vi "Stewart_platform_6_deg_freedom_ver4_easier_upgrade.vi"() -> ()   [LabVIEW 2019]
uses:
  SubVI/Type_definition_updated_motion_output_row.ctl
  SubVI/Type_definition_current_motion.ctl
  SubVI/Type_definition.ctl
panel:
  out "結果":bool
  in  "One way control":T1={"T"=2000.0, "Linear or sine?"=0.0, "Buffer size"=0.5, "Buffer power"=3.0}
  out "Default output":T2
  out "YZcirc output":T2
  in  "YZcirc control":T3={"YZcirc Initial State"=[[0.0], [0.0], [0.0], [0.0], [0.0], [220.0]], "gamma1"=240.0, "T"=4000.0, "One or negative one"=1.0}
  out "Zvert output":T2
  in  "Zvert control":T4={"Zvert Initial State"=[[0.0], [0.0], [0.0], [0.0], [0.0], [240.0]], "gamma1"=220.0, "T"=4000.0}
  in  "Bytes at buffer":u32
  in  "Sample rate":dbl
  in  "Decoder main":i32[](array[numeric])
  in  "Stop ALL":bool=TRUE
  out "XYZrot output":T2
  out "Tau output":T2
  out "Tilt output":T2
  out "Rot output":T2
  in  "Motion Selector":T5
  in  "TERMINATE":bool
  in  "Iteration count":i32
  in  "Current Motion":T6
  in  "Sampled current position":dbl[](array[numeric])
  out "Rawoffset":dbl[][](array[numeric])
  out "Updated Motion Output Row":T7
  in  "Instant Start / Stop":bool
  in  "Feedback enabled?":bool
  in  "Start / Stop after cycle completion":bool
  out "One way output":T2
  in  "Default Position":T8={"Rot Initial State"=[[0.0], [0.0], [0.0], [0.0], [0.0], [230.0]], "One or negative one"=1.0, "T"=5000.0}
  in  "XYZrot control":T9={"XYZ Initial State"=[[0.0], [0.0], [0.0], [20.0], [0.0], [230.0]], "One or negative one"=1.0, "T"=4000.0}
  in  "Tau control":T10={"Tau Initial State"=[[0.0], [0.0], [15.0], [0.0], [0.0], [230.0]], "One or negative one"=1.0, "T"=4000.0}
  in  "Tilt control":T11={"Tilt Initial State"=[[90.0], [10.0], [0.0], [0.0], [0.0], [230.0]], "One or negative one"=1.0, "T"=4000.0}
  in  "Rot control":T8={"Rot Initial State"=[[0.0], [10.0], [0.0], [0.0], [0.0], [230.0]], "One or negative one"=1.0, "T"=4000.0}
  out "Achievable?":errorcluster caption="s? t:f"
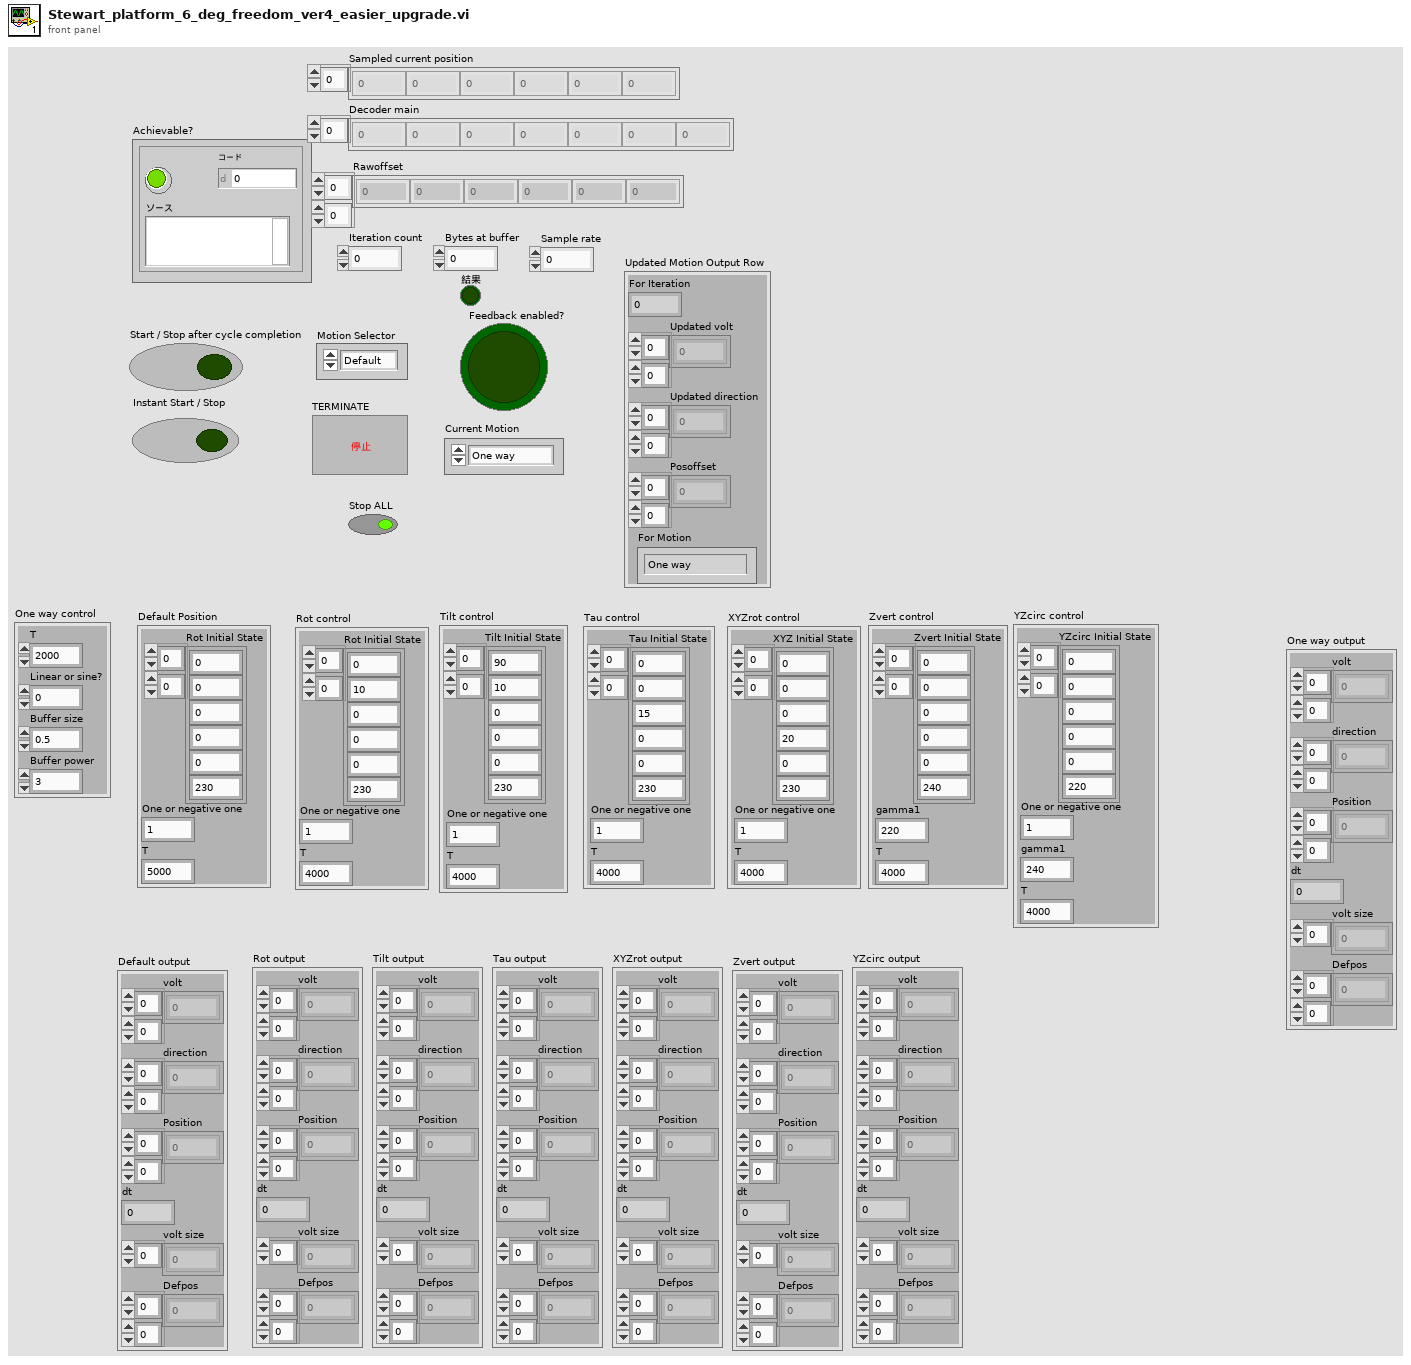
[diagram p1: front panel]
types:
  T1 = cluster{"T":dbl, "Linear or sine?":dbl, "Buffer size":dbl, "Buffer power":dbl}
  T2 = cluster{"volt":dbl[][], "direction":dbl[][], "Position":dbl[][], "dt":dbl, "volt size":i32[], "Defpos":dbl[][]}
  T3 = cluster{"YZcirc Initial State":dbl[][], "gamma1":dbl, "T":dbl, "One or negative one":dbl}
  T4 = cluster{"Zvert Initial State":dbl[][], "gamma1":dbl, "T":dbl}
  T5 = typedef "Type_definition.ctl" = enum16{"Default", "Rot", "Tilt", "Tau", "XYZrot", "Zvert", "YZcirc"}
  T6 = typedef "Type_definition_current_motion.ctl" = enum16{"One way", "Rot", "Tilt", "Tau", "XYZrot", "Zvert", "YZcirc", "Random direction tilt"}
  T7 = typedef "Type_definition_updated_motion_output_row.ctl" = cluster{"For Iteration":dbl, "Updated volt":dbl[][], "Updated direction":dbl[][], "Posoffset":dbl[][], "For Motion":T6}
  T8 = cluster{"Rot Initial State":dbl[][], "One or negative one":dbl, "T":dbl}
  T9 = cluster{"XYZ Initial State":dbl[][], "One or negative one":dbl, "T":dbl}
  T10 = cluster{"Tau Initial State":dbl[][], "One or negative one":dbl, "T":dbl}
  T11 = cluster{"Tilt Initial State":dbl[][], "One or negative one":dbl, "T":dbl}
  T12 = cluster{"Default State":dbl[][], "Rot Initial State":dbl[][], "Tilt Initial State":dbl[][], "Tau Initial State":dbl[][], "XYZrot Initial State":dbl[][], "Zvert Initial State":dbl[][], "YZcirc Initial State":dbl[][]}
  T13 = cluster{"Rot output":cluster{"volt":dbl[][], "direction":dbl[][], "Position":dbl[][], "dt":dbl, "volt size":i32[], "Defpos":dbl[][]}, "Tilt output":cluster{"volt":dbl[][], "direction":dbl[][], "Position":dbl[][], "dt":dbl, "volt size":i32[], "Defpos":dbl[][]}, "Tau output":cluster{"volt":dbl[][], "direction":dbl[][], "Position":dbl[][], "dt":dbl, "volt size":i32[], "Defpos":dbl[][]}, "XYZrot output":cluster{"volt":dbl[][], "direction":dbl[][], "Position":dbl[][], "dt":dbl, "volt size":i32[], "Defpos":dbl[][]}, "Default output":cluster{"volt":dbl[][], "direction":dbl[][], "Position":dbl[][], "dt":dbl, "volt size":i32[], "Defpos":dbl[][]}, "Zvert Output":cluster{"volt":dbl[][], "direction":dbl[][], "Position":dbl[][], "dt":dbl, "volt size":i32[], "Defpos":dbl[][]}, "YZcirc Output":cluster{"volt":dbl[][], "direction":dbl[][], "Position":dbl[][], "dt":dbl, "volt size":i32[], "Defpos":dbl[][]}}
  T14 = enum8{"Enabled", "Disabled", "Disabled and Grayed Out"}
  T15 = cluster{"Achievable":dbl, "TT":dbl, "tt":dbl, "dt":dbl, "pulserev":dbl, "distrev":dbl, "ArdNI_ratio":dbl, "A":dbl, "B":dbl, "qmax":dbl, "qmin":dbl, "q0":dbl[][], "r":dbl, "ballangle":dbl[][], "diskofst":dbl, "l":dbl[][], "L":dbl}
  T16 = cluster{"theta":dbl[][], "phi":dbl[][], "tau":dbl[][], "p":dbl[][], "T":dbl}
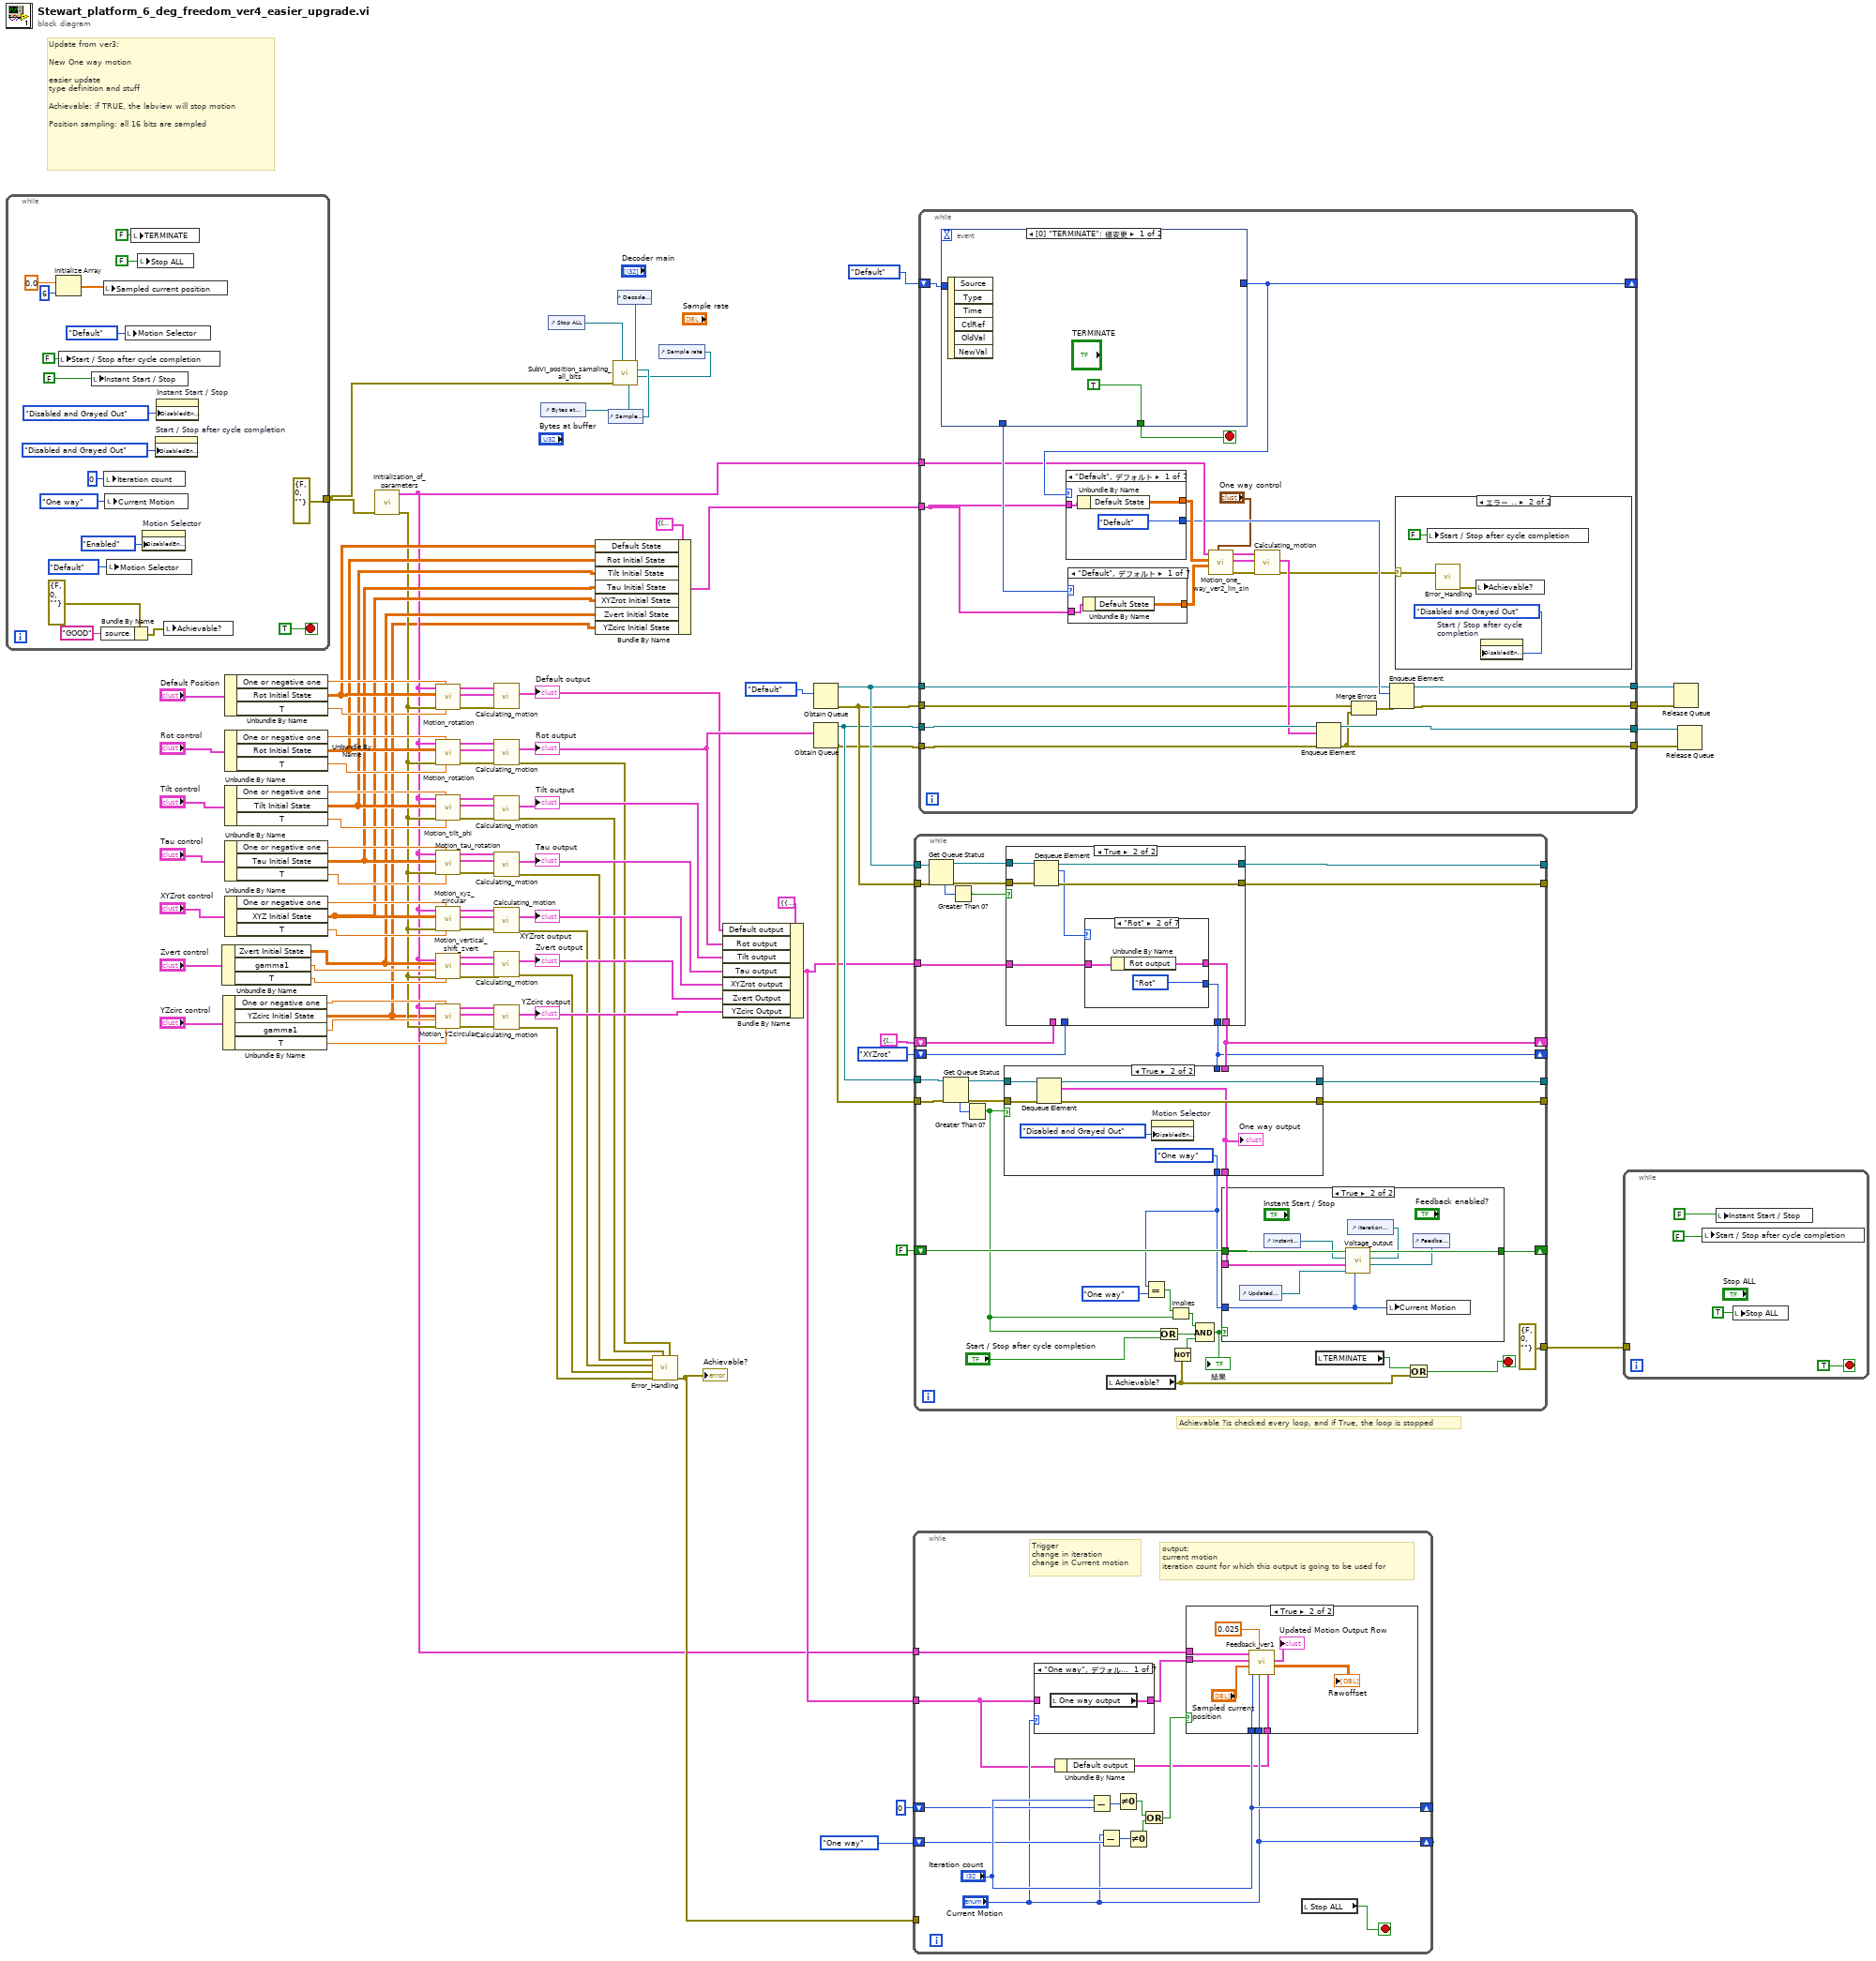
[diagram p0: block diagram]
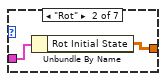
[diagram p3: hidden frame]
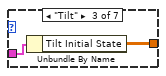
[diagram p4: hidden frame]
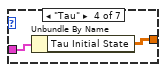
[diagram p5: hidden frame]
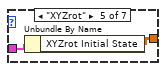
[diagram p6: hidden frame]
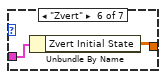
[diagram p7: hidden frame]
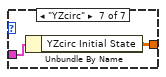
[diagram p8: hidden frame]
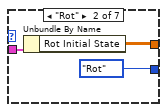
[diagram p9: hidden frame]
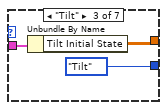
[diagram p10: hidden frame]
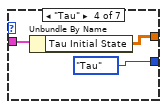
[diagram p11: hidden frame]
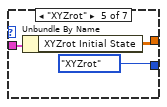
[diagram p12: hidden frame]
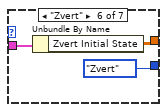
[diagram p13: hidden frame]
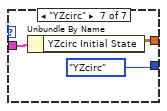
[diagram p14: hidden frame]
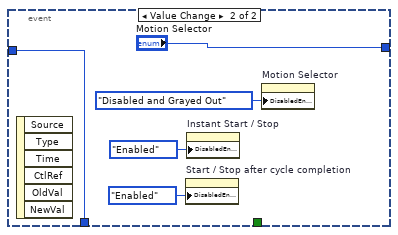
[diagram p15: hidden frame]
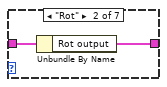
[diagram p16: hidden frame]
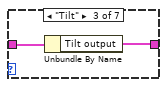
[diagram p17: hidden frame]
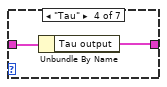
[diagram p18: hidden frame]
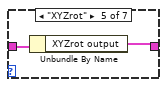
[diagram p19: hidden frame]
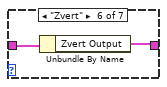
[diagram p20: hidden frame]
diagram:
  # "Achievable ?is checked every loop, and if True, the loop is stopped"
  # "Update from ver3:\n\nNew One way motion\n \neasier update\ntype definition and stuff\n\nAchievable: if TRUE, the labview will stop motion\n\nPosition sampling: all 16 bits are sampled"
  n1 = while {
    tunnel: [errorcluster {"status"=FALSE, "code"=0, "source"=""} ("エラー定数")] -> w6
    stop <- TRUE stop-if-true
    n2 = Initialize Array(0.0, 6 ("次元サイズ")) -> (w96:dbl[])
    n3 = local write "Start / Stop after cycle completion"(FALSE ("Terminate")) -> ()
    n4 = local write "Instant Start / Stop"(FALSE ("Terminate")) -> ()
    n5 = Bundle By Name(cluster=errorcluster {"status"=FALSE, "code"=0, "source"=""} ("エラー定数"), "source"="GOOD") -> (w93:errorcluster)
    n6 = local write "Sampled current position"(w96) -> ()
    n7 = local write "Iteration count"(0 ("Iteration count")) -> ()
    n8 = local write "Current Motion"(Type_definition_current_motion."One way" ("Current Motion")) -> ()
    n9 = local write "Motion Selector"(Type_definition."Default" ("Motion Selector")) -> ()
    n10 = local write "Motion Selector"(Type_definition."Default" ("Motion Selector")) -> ()
    n11 = local write "TERMINATE"(FALSE ("Terminate")) -> ()
    n12 = local write "Stop ALL"(FALSE ("Terminate")) -> ()
    n13 = property on="Motion Selector" class="Enum (指定)"("DisabledEnum"=T14."Enabled" ("無効")) -> ()  [unwired: 2 in, 2 out]
    n14 = property on="Start / Stop after cycle completion" class="Bool (指定)"("DisabledEnum"=T14."Disabled and Grayed Out" ("無効")) -> ()  [unwired: 2 in, 2 out]
    n15 = property on="Instant Start / Stop" class="Bool (指定)"("DisabledEnum"=T14."Disabled and Grayed Out" ("無効")) -> ()  [unwired: 2 in, 2 out]
    n16 = local write "Achievable?"(w93) -> ()
  }
  n17 = Unbundle By Name("Zvert control") -> ("Zvert Initial State"=w24:dbl[][], "gamma1"=w27:dbl, "T"=w26:dbl)
  n18 = Unbundle By Name("YZcirc control") -> ("One or negative one"=w22:dbl, "YZcirc Initial State"=w7:dbl[][], "gamma1"=w21:dbl, "T"=w20:dbl)
  n19 = Unbundle By Name("Default Position") -> ("One or negative one"=w67:dbl, "Rot Initial State"=w59:dbl[][], "T"=w68:dbl)
  n20 = Unbundle By Name("Rot control") -> ("One or negative one"=w79:dbl, "Rot Initial State"=w58:dbl[][], "T"=w78:dbl)
  n21 = Unbundle By Name("Tilt control") -> ("One or negative one"=w76:dbl, "Tilt Initial State"=w57:dbl[][], "T"=w75:dbl)
  n22 = Unbundle By Name("Tau control") -> ("One or negative one"=w73:dbl, "Tau Initial State"=w56:dbl[][], "T"=w72:dbl)
  n23 = Unbundle By Name("XYZrot control") -> ("One or negative one"=w70:dbl, "XYZ Initial State"=w55:dbl[][], "T"=w69:dbl)
  n24 = call "Initialization_of_parameters.vi"("Error IN"=w6) -> ("Error OUT"=w19:errorcluster, "Initial constants"=w14:T15)  [unwired: 8 in]
  n25 = call "Motion_rotation.vi"("T"=w68, "One_or_negativeone"=w67, "Error IN"=w19, "Initial State"=w59, "Constants IN"=w14) -> ("Error OUT"=w65:errorcluster, "Motion sequence"=w61:T16, "Constants OUT"=w64:T15)  [unwired: 4 in]
  n26 = call "Motion_rotation.vi"("T"=w78, "One_or_negativeone"=w79, "Error IN"=w19, "Initial State"=w58, "Constants IN"=w14) -> ("Error OUT"=w90:errorcluster, "Motion sequence"=w91:T16, "Constants OUT"=w92:T15)  [unwired: 4 in]
  n27 = call "Motion_tilt_phi.vi"("T"=w75, "One_or_negativeone"=w76, "Error IN"=w19, "Initial State"=w57, "Constants IN"=w14) -> ("Error OUT"=w87:errorcluster, "Motion Sequence"=w88:T16, "Constants OUT"=w89:T15)  [unwired: 4 in]
  n28 = call "Motion_tau_rotation.vi"("T"=w72, "One_or_negativeone"=w73, "Error IN"=w19, "Initial State"=w56, "Constants IN"=w14) -> ("Error OUT"=w84:errorcluster, "Motion Sequence"=w85:T16, "Constants OUT"=w86:T15)  [unwired: 4 in]
  n29 = call "Motion_xyz_circular.vi"("T"=w69, "One_or_negativeone"=w70, "Error IN"=w19, "Initial State"=w55, "Constants IN"=w14) -> ("Error OUT"=w81:errorcluster, "Motion Sequence"=w82:T16, "Constants OUT"=w83:T15)  [unwired: 4 in]
  n30 = call "Motion_vertical_shift_zvert.vi"("T"=w26, "Error IN"=w19, "gamma1"=w27, "Initial State"=w24, "Constants IN"=w14) -> ("Error OUT"=w29:errorcluster, "Motion sequence"=w30:T16, "Constants OUT"=w31:T15)  [unwired: 4 in]
  n31 = call "Motion_YZcircular.vi"("T"=w20, "One_or_negativeone"=w22, "Error IN"=w19, "gamma1"=w21, "Initial State"=w7, "Constants IN"=w14) -> ("Error OUT"=w17:errorcluster, "Motion Sequence"=w16:T16, "Constants OUT"=w18:T15)  [unwired: 3 in]
  n32 = call "Calculating_motion.vi"("Error IN"=w65, "Motion sequence"=w61, "Constants IN"=w64) -> ("Output"=w32:T2)  [unwired: 6 in, 2 out]
  "Default output" <- w32
  n33 = call "Calculating_motion.vi"("Error IN"=w90, "Motion sequence"=w91, "Constants IN"=w92) -> ("Error OUT"=w13:errorcluster, "Output"=w41:T2)  [unwired: 6 in, 1 out]
  "Rot output" <- w41
  n34 = call "Calculating_motion.vi"("Error IN"=w87, "Motion sequence"=w88, "Constants IN"=w89) -> ("Error OUT"=w12:errorcluster, "Output"=w40:T2)  [unwired: 6 in, 1 out]
  "Tilt output" <- w40
  n35 = call "Calculating_motion.vi"("Error IN"=w84, "Motion sequence"=w85, "Constants IN"=w86) -> ("Error OUT"=w11:errorcluster, "Output"=w39:T2)  [unwired: 6 in, 1 out]
  "Tau output" <- w39
  n36 = call "Calculating_motion.vi"("Error IN"=w81, "Motion sequence"=w82, "Constants IN"=w83) -> ("Error OUT"=w10:errorcluster, "Output"=w38:T2)  [unwired: 6 in, 1 out]
  "XYZrot output" <- w38
  n37 = call "Calculating_motion.vi"("Error IN"=w29, "Motion sequence"=w30, "Constants IN"=w31) -> ("Error OUT"=w9:errorcluster, "Output"=w25:T2)  [unwired: 6 in, 1 out]
  "Zvert output" <- w25
  n38 = call "Calculating_motion.vi"("Error IN"=w17, "Motion sequence"=w16, "Constants IN"=w18) -> ("Error OUT"=w8:errorcluster, "Output"=w15:T2)  [unwired: 6 in, 1 out]
  "YZcirc output" <- w15
  n39 = control-ref of="Bytes at buffer"() -> (w33:refnum<vi>)
  n40 = control-ref of="Stop ALL"() -> (w36:refnum<vi>)
  n41 = Bundle By Name(cluster=T12 {"Default State"=[], "Rot Initial State"=[], "Tilt Initial State"=[], "Tau Initial State"=[], "XYZrot Initial State"=[], "Zvert Initial State"=[], "YZcirc Initial State"=[]}, "Default State"=w59, "Rot Initial State"=w58, "Tilt Initial State"=w57, "Tau Initial State"=w56, "XYZrot Initial State"=w55, "Zvert Initial State"=w24, "YZcirc Initial State"=w7) -> (w54:T12)
  n42 = control-ref of="Sampled current position"() -> (w43:refnum<vi>)
  n43 = control-ref of="Decoder main"() -> (w35:refnum<vi>)
  n44 = call "Error_Handling.vi"("1"=w13, "2"=w12, "6"=w8, "5"=w9, "4"=w10, "3"=w11) -> ("Error OUT"=w62:errorcluster)  [unwired: 5 in]
  "Achievable?" <- w62
  n45 = control-ref of="Sample rate"() -> (w34:refnum<vi>)
  n46 = call "SubVI_position_sampling_all_bits.vi"("Sample rate"=w34, "Sampled current position"=w43, "Decoder main"=w35, "Bytes at buffer"=w33, "Stop ALL"=w36, "Error IN (no error)"=w6) -> ()  [unwired: 5 in, 1 out]
  n47 = Bundle By Name(cluster=T13 {"Rot output"={"volt"=[], "direction"=[], "Position"=[], "dt"=0.0, "volt size"=[], "Defpos"=[]}, "Tilt output"={"volt"=[], "direction"=[], "Position"=[], "dt"=0.0, "volt size"=[], "Defpos"=[]}, "Tau output"={"volt"=[], "direction"=[], "Position"=[], "dt"=0.0, "volt size"=[], "Defpos"=[]}, "XYZrot output"={"volt"=[], "direction"=[], "Position"=[], "dt"=0.0, "volt size"=[], "Defpos"=[]}, "Default output"={"volt"=[], "direction"=[], "Position"=[], "dt"=0.0, "volt size"=[], "Defpos"=[]}, "Zvert Output"={"volt"=[], "direction"=[], "Position"=[], "dt"=0.0, "volt size"=[], "Defpos"=[]}, "YZcirc Output"={"volt"=[], "direction"=[], "Position"=[], "dt"=0.0, "volt size"=[], "Defpos"=[]}}, "Default output"=w32, "Rot output"=w41, "Tilt output"=w40, "Tau output"=w39, "XYZrot output"=w38, "Zvert Output"=w25, "YZcirc Output"=w15) -> (w45:T13)
  n48 = Obtain Queue(element data type=Type_definition."Default" ("Motion Selector")) -> (queue out=w52:refnum<queue>, error out=w51:errorcluster)  [unwired: 4 in, 1 out]
  n49 = Obtain Queue(element data type=w41) -> (queue out=w50:refnum<queue>, error out=w49:errorcluster)  [unwired: 4 in, 1 out]
  n50 = while {
    tunnel: w14 -> [w125]
    shift-right: ["Iteration count"] -> _
    shift-left: 0 ("Iteration count") -> [w123]
    shift-right: ["Current Motion"] -> _
    shift-left: Type_definition_current_motion."One way" ("Current Motion") -> [w122]
    tunnel: w62 -> [_]
    tunnel: w45 -> [w113]
    stop <- w114 stop-if-true
    # "Trigger\nchange in iteration\nchange in Current motion"
    # "output:\ncurrent motion\niteration count for which this output is going to be used for"
    n51 = case shown="\"One way\", デフォルト" "Current Motion" {
      tunnel: w113 -> [_ w128 w130 w132 w134 w136 w138]
      tunnel: [w126 w127 w129 w131 w133 w135 w137] -> w115
      frame "One way", Default {
        n52 = local read "One way output"() -> (w126:T2)
      }
      frame "Rot" {
        n53 = Unbundle By Name(w128) -> ("Rot output"=w127:T2)
      }
      frame "Tilt" {
        n54 = Unbundle By Name(w130) -> ("Tilt output"=w129:T2)
      }
      frame "Tau" {
        n55 = Unbundle By Name(w132) -> ("Tau output"=w131:T2)
      }
      frame "XYZrot" {
        n56 = Unbundle By Name(w134) -> ("XYZrot output"=w133:T2)
      }
      frame "Zvert" {
        n57 = Unbundle By Name(w136) -> ("Zvert Output"=w135:T2)
      }
      frame "YZcirc" {
        n58 = Unbundle By Name(w138) -> ("YZcirc Output"=w137:T2)
      }
    }
    n59 = Unbundle By Name(w113) -> ("Default output"=w112:T2)
    n60 = Subtract(x="Iteration count", y=w123) -> (x-y=w121:i32)
    n61 = Subtract(x="Current Motion", y=w122) -> (x-y=w120:u16)
    n62 = Not Equal To 0?(x=w121) -> (x != 0?=w118:bool)
    n63 = Not Equal To 0?(x=w120) -> (x != 0?=w119:bool)
    n64 = Or(x=w118, y=w119) -> (x .or. y?=w117:bool)
    n65 = case shown="TRUE" w117 {
      tunnel: "Iteration count" -> [_ w147]
      tunnel: w125 -> [_ w146]
      tunnel: "Current Motion" -> [_ w143]
      tunnel: w115 -> [_ w141]
      tunnel: w112 -> [_ w139]
      frame False {
      }
      frame True {
        n66 = call "Feedback_ver1.vi"("Default output"=w139, "Current Motion"=w143, "bound"=0.025, "Iteration"=w147, "Sampled current position"="Sampled current position", "Current Motion Output"=w141, "Initial constants"=w146) -> ("Rawoffset"=→"Rawoffset":dbl[][], "Updated Motion Output Row"=→"Updated Motion Output Row":T7)  [unwired: 3 in]
      }
    }
    n67 = local read "Stop ALL"() -> (w114:bool)
  }
  n68 = while {
    shift-right: [w183] -> _
    shift-left: FALSE ("Toggle OUT") -> [w182]
    tunnel: w52 -> [w181]
    tunnel: w51 -> [w180]
    tunnel: [w175] -> _
    tunnel: [w174] -> _
    tunnel: w50 -> [w168]
    tunnel: w49 -> [w167]
    tunnel: [w173] -> _
    tunnel: [w172] -> _
    tunnel: w45 -> [w171]
    shift-right: [w164] -> _
    shift-left: T2 {"volt"=[], "direction"=[], "Position"=[], "dt"=0.0, "volt size"=[], "Defpos"=[]} ("Output") -> [w170]
    shift-right: [w160] -> _
    shift-left: Type_definition_current_motion."XYZrot" ("Current Motion") -> [w161]
    tunnel: [errorcluster {"status"=FALSE, "code"=0, "source"=""} ("エラー定数")] -> w37
    stop <- w153 stop-if-true
    n69 = Get Queue Status(queue=w181, error in (no error)=w180) -> (queue out=w176:refnum<queue>, error out=w177:errorcluster, # elements in queue=w179:i32)  [unwired: 1 in, 5 out]
    n70 = Get Queue Status(queue=w168, error in (no error)=w167) -> (queue out=w166:refnum<queue>, error out=w165:errorcluster, # elements in queue=w169:i32)  [unwired: 1 in, 5 out]
    n71 = Greater Than 0?(x=w179) -> (x > 0?=w178:bool)
    n72 = Greater Than 0?(x=w169) -> (x > 0?=w159:bool)
    n73 = case shown="TRUE" w178 {
      tunnel: w177 -> [w198 w207]
      tunnel: w176 -> [w199 w206]
      tunnel: [w199 w205] -> w175
      tunnel: [w198 w204] -> w174
      tunnel: w171 -> [_ w203]
      tunnel: [w197 w201] -> w164
      tunnel: w170 -> [w197 _]
      tunnel: [w196 w200] -> w160
      tunnel: w161 -> [w196 _]
      frame False {
      }
      frame True {
        n74 = Dequeue Element(queue=w206, error in (no error)=w207) -> (queue out=w205:refnum<queue>, element=w202:T5, error out=w204:errorcluster)  [unwired: 1 in, 1 out]
        n75 = case shown="\"Rot\"" w202 {
          tunnel: w203 -> [w210 w213 w216 w219 w222 w225 w228]
          tunnel: [w209 w212 w215 w218 w221 w224 w227] -> w201
          tunnel: [Type_definition_current_motion."One way" ("Current Motion") Type_definition_current_motion."Rot" ("Current Motion") Type_definition_current_motion."Tilt" ("Current Motion") Type_definition_current_motion."Tau" ("Current Motion") Type_definition_current_motion."XYZrot" ("Current Motion") Type_definition_current_motion."Zvert" ("Current Motion") Type_definition_current_motion."YZcirc" ("Current Motion")] -> w200
          frame "Default", Default {
            n76 = Unbundle By Name(w210) -> ("Rot output"=w209:T2)
          }
          frame "Rot" {
            n77 = Unbundle By Name(w213) -> ("Rot output"=w212:T2)
          }
          frame "Tilt" {
            n78 = Unbundle By Name(w216) -> ("Tilt output"=w215:T2)
          }
          frame "Tau" {
            n79 = Unbundle By Name(w219) -> ("Tau output"=w218:T2)
          }
          frame "XYZrot" {
            n80 = Unbundle By Name(w222) -> ("XYZrot output"=w221:T2)
          }
          frame "Zvert" {
            n81 = Unbundle By Name(w225) -> ("Zvert Output"=w224:T2)
          }
          frame "YZcirc" {
            n82 = Unbundle By Name(w228) -> ("YZcirc Output"=w227:T2)
          }
        }
      }
    }
    n83 = case shown="TRUE" w159 {
      tunnel: [w188 w195] -> w173
      tunnel: [w187 w194] -> w172
      tunnel: w166 -> [w188 w193]
      tunnel: w165 -> [w187 w192]
      tunnel: w164 -> [w186 _]
      tunnel: [w186 w189] -> w163
      tunnel: w160 -> [w184 _]
      tunnel: [w184 Type_definition_current_motion."One way" ("Current Motion")] -> w155
      frame False {
        n84 = property on="Motion Selector" class="Enum (指定)"("DisabledEnum"=T14."Enabled" ("無効")) -> ()  [unwired: 2 in, 2 out]
      }
      frame True {
        n85 = Dequeue Element(queue=w193, error in (no error)=w192) -> (queue out=w195:refnum<queue>, element=w189:T2, error out=w194:errorcluster)  [unwired: 1 in, 1 out]
        "One way output" <- w189
        n86 = property on="Motion Selector" class="Enum (指定)"("DisabledEnum"=T14."Disabled and Grayed Out" ("無効")) -> ()  [unwired: 2 in, 2 out]
      }
    }
    n87 = local read "Achievable?"() -> (w149:errorcluster)
    n88 = Equal?(x=w155, y=Type_definition_current_motion."One way" ("Current Motion")) -> (x = y?=w158:bool)
    n89 = Or(x=w159, y="Start / Stop after cycle completion") -> (x .or. y?=w150:bool)
    n90 = Implies(1:w159, 2:w158) -> (0:w152:bool)
    n91 = Not(x=w149) -> (.not. x?=w148:bool)
    n92 = Compound Arithmetic op=AND ("複合演算")(w152, w150, w148) -> (w151:bool)
    "結果" <- w151
    n93 = case shown="TRUE" w151 {
      tunnel: [w230 w238] -> w183
      tunnel: w182 -> [w230 w237]
      tunnel: w163 -> [_ w236]
      tunnel: w155 -> [_ w235]
      frame False {
        n94 = local write "Instant Start / Stop"(FALSE) -> ()
      }
      frame True {
        n95 = control-ref of="Updated Motion Output Row"() -> (w231:refnum<vi>)
        n96 = control-ref of="Instant Start / Stop"() -> (w234:refnum<vi>)
        n97 = control-ref of="Iteration count"() -> (w233:refnum<vi>)
        n98 = local write "Current Motion"(w235) -> ()
        n99 = control-ref of="Feedback enabled?"() -> (w232:refnum<vi>)
        n100 = call "Voltage_output.vi"("Feedback enabled?"=w232, "Iteration count"=w233, "Current Motion"=w235, "Updated Motion Output Row"=w231, "Current Motion Output"=w236, "Instant Start / Stop"=w234, "Toggle IN"=w237) -> ("Toggle OUT"=w238:bool)  [unwired: 4 in]
      }
    }
    n101 = local read "TERMINATE"() -> (w154:bool)
    n102 = Or(x=w154, y=w149) -> (x .or. y?=w153:bool)
  }
  n103 = while {
    shift-right: [w260] -> _
    shift-left: Type_definition."Default" ("Motion Selector") -> [w261]
    tunnel: w54 -> [w258]
    tunnel: w14 -> [w255]
    tunnel: w50 -> [w254]
    tunnel: w49 -> [w253]
    tunnel: w52 -> [w245]
    tunnel: w51 -> [w244]
    tunnel: [w248] -> w5
    tunnel: [w247] -> w4
    tunnel: [w246] -> w3
    tunnel: [w243] -> w2
    stop <- w262 stop-if-true
    n104 = event shown="[0] \"TERMINATE\": 値変更" {
      selector: _ -> [_ _]
      dyn-events: _ -> [_ _]
      timeout: _ -> [_ _]
      tunnel: [TRUE _] -> w262
      tunnel: w261 -> [_ w307]
      tunnel: [_ "Motion Selector"] -> w260
      tunnel: [_ w307] -> w259
      event "TERMINATE": Value Change {
        n105 = event-data() -> ()  [unwired: 1 in, 6 out]
      }
      event Value Change {
        n106 = event-data() -> ()  [unwired: 1 in, 6 out]
        n107 = property on="Start / Stop after cycle completion" class="Bool (指定)"("DisabledEnum"=T14."Enabled" ("無効")) -> ()  [unwired: 2 in, 2 out]
        n108 = property on="Instant Start / Stop" class="Bool (指定)"("DisabledEnum"=T14."Enabled" ("無効")) -> ()  [unwired: 2 in, 2 out]
        n109 = property on="Motion Selector" class="Enum (指定)"("DisabledEnum"=T14."Disabled and Grayed Out" ("無効")) -> ()  [unwired: 2 in, 2 out]
      }
    }
    n110 = case shown="\"Default\", デフォルト" w260 {
      tunnel: w258 -> [w283 w286 w289 w292 w295 w298 w300]
      tunnel: [w282 w285 w288 w291 w294 w296 w299] -> w257
      tunnel: [Type_definition."Default" ("Motion Selector") Type_definition."Rot" ("Motion Selector") Type_definition."Tilt" ("Motion Selector") Type_definition."Tau" ("Motion Selector") Type_definition."XYZrot" ("Motion Selector") Type_definition."Zvert" ("Motion Selector") Type_definition."YZcirc" ("Motion Selector")] -> w249
      frame "Default", Default {
        n111 = Unbundle By Name(w283) -> ("Default State"=w282:dbl[][])
      }
      frame "Rot" {
        n112 = Unbundle By Name(w286) -> ("Rot Initial State"=w285:dbl[][])
      }
      frame "Tilt" {
        n113 = Unbundle By Name(w289) -> ("Tilt Initial State"=w288:dbl[][])
      }
      frame "Tau" {
        n114 = Unbundle By Name(w292) -> ("Tau Initial State"=w291:dbl[][])
      }
      frame "XYZrot" {
        n115 = Unbundle By Name(w295) -> ("XYZrot Initial State"=w294:dbl[][])
      }
      frame "Zvert" {
        n116 = Unbundle By Name(w298) -> ("Zvert Initial State"=w296:dbl[][])
      }
      frame "YZcirc" {
        n117 = Unbundle By Name(w300) -> ("YZcirc Initial State"=w299:dbl[][])
      }
    }
    n118 = case shown="\"Default\", デフォルト" w259 {
      tunnel: w258 -> [w268 w270 w272 w274 w276 w278 w280]
      tunnel: [w267 w269 w271 w273 w275 w277 w279] -> w256
      frame "Default", Default {
        n119 = Unbundle By Name(w268) -> ("Default State"=w267:dbl[][])
      }
      frame "Rot" {
        n120 = Unbundle By Name(w270) -> ("Rot Initial State"=w269:dbl[][])
      }
      frame "Tilt" {
        n121 = Unbundle By Name(w272) -> ("Tilt Initial State"=w271:dbl[][])
      }
      frame "Tau" {
        n122 = Unbundle By Name(w274) -> ("Tau Initial State"=w273:dbl[][])
      }
      frame "XYZrot" {
        n123 = Unbundle By Name(w276) -> ("XYZrot Initial State"=w275:dbl[][])
      }
      frame "Zvert" {
        n124 = Unbundle By Name(w278) -> ("Zvert Initial State"=w277:dbl[][])
      }
      frame "YZcirc" {
        n125 = Unbundle By Name(w280) -> ("YZcirc Initial State"=w279:dbl[][])
      }
    }
    n126 = call "Motion_one_way_ver2_lin_sin.vi"("Parameters"="One way control", "previousSTATE"=w256, "nextSTATE"=w257, "Constants IN"=w255) -> ("Error OUT"=w252:errorcluster, "Motion Sequence"=w240:T16, "Constants OUT"=w251:T15)  [unwired: 5 in]
    n127 = call "Calculating_motion.vi"("Error IN"=w252, "Motion sequence"=w240, "Constants IN"=w251) -> ("Error OUT"=w241:errorcluster, "Output"=w250:T2)  [unwired: 6 in, 1 out]
    n128 = Enqueue Element(queue=w254, element=w250, error in (no error)=w253) -> (queue out=w246:refnum<queue>, error out=w243:errorcluster)  [unwired: 1 in, 1 out]
    n129 = Merge Errors(w244, w243) -> (w242:errorcluster)
    n130 = Enqueue Element(queue=w245, element=w249, error in (no error)=w242) -> (queue out=w248:refnum<queue>, error out=w247:errorcluster)  [unwired: 1 in, 1 out]
    n131 = case shown="エラー .." w241 {
      selector: w241 -> [_ w266]
      frame No Error {
      }
      frame Error {
        n132 = local write "Start / Stop after cycle completion"(FALSE ("Instant Start / Stop")) -> ()
        n133 = call "Error_Handling.vi"("4"=w266) -> ("Error OUT"=w263:errorcluster)  [unwired: 10 in]
        n134 = local write "Achievable?"(w263) -> ()
        n135 = property on="Start / Stop after cycle completion" class="Bool (指定)"("DisabledEnum"=T14."Disabled and Grayed Out" ("無効")) -> ()  [unwired: 2 in, 2 out]
      }
    }
  }
  n136 = while {
    tunnel: w37 -> [_]
    stop <- TRUE stop-if-true
    n137 = local write "Start / Stop after cycle completion"(FALSE ("STOP ALL")) -> ()
    n138 = local write "Instant Start / Stop"(FALSE ("STOP ALL")) -> ()
    n139 = local write "Stop ALL"(TRUE ("STOP ALL")) -> ()
  }
  n140 = Release Queue(queue=w5, error in (no error)=w4) -> ()  [unwired: 1 in, 3 out]
  n141 = Release Queue(queue=w3, error in (no error)=w2) -> ()  [unwired: 1 in, 3 out]
